vi "Diff_Drive_System_Act.vi"(6 "FPGA_Time_Seconds":dbl, 7 "Enabled":bool=TRUE, 9 "Right Speed":dbl, 10 "Left Speed":dbl, 11 "Diff_Drive_Device_Refs":T1 {"GyroDevRef"."Sample Rate" min=0.25 max=100.0 step=0.25}) -> ()   [LabVIEW 2019]
uses:
  <vilib>/Rock Robotics/WPI/ThirdParty/JAS_Junk/TrajLib/Trajectory_Library.lvlib
  Diff_Drive_System_Globals.vi
  <vilib>/Rock Robotics/SystemInterfaces/DIO/FPGA_DIOPWMChannel.ctl
  <vilib>/Rock Robotics/WPI/PWM/WPI_PWMDeadband.ctl
  <vilib>/Rock Robotics/WPI/MotorControl/WPI_MotorControlType.ctl
  <vilib>/Rock Robotics/SystemInterfaces/DIO/FPGA_DIOChannel.ctl
  <vilib>/Rock Robotics/WPI/MotorControl/WPI_MotorControlDeviceRef.ctl
  <vilib>/Rock Robotics/WPI/RobotDrive/WPI_RobotDriveDevRef.ctl
  <vilib>/Rock Robotics/SystemInterfaces/Encoder/FPGA_EncoderIdx.ctl
  <vilib>/Rock Robotics/WPI/Encoder/WPI_EncoderType.ctl
  <vilib>/Rock Robotics/SystemInterfaces/Counter/FPGA_CounterCtrSystemIndex.ctl
  <vilib>/Rock Robotics/WPI/Encoder/WPI_EncoderDevRef.ctl
  <vilib>/Rock Robotics/SystemInterfaces/spilib/spi_bus.ctl
  <vilib>/Rock Robotics/SystemInterfaces/AI/FPGA_AIChannel.ctl
  <vilib>/Rock Robotics/WPI/Gyro/WPI_GyroDevRef.ctl
  Diff_Drive_System_Device_Refs.ctl
panel:
  # "Analog"
  # "XRS"
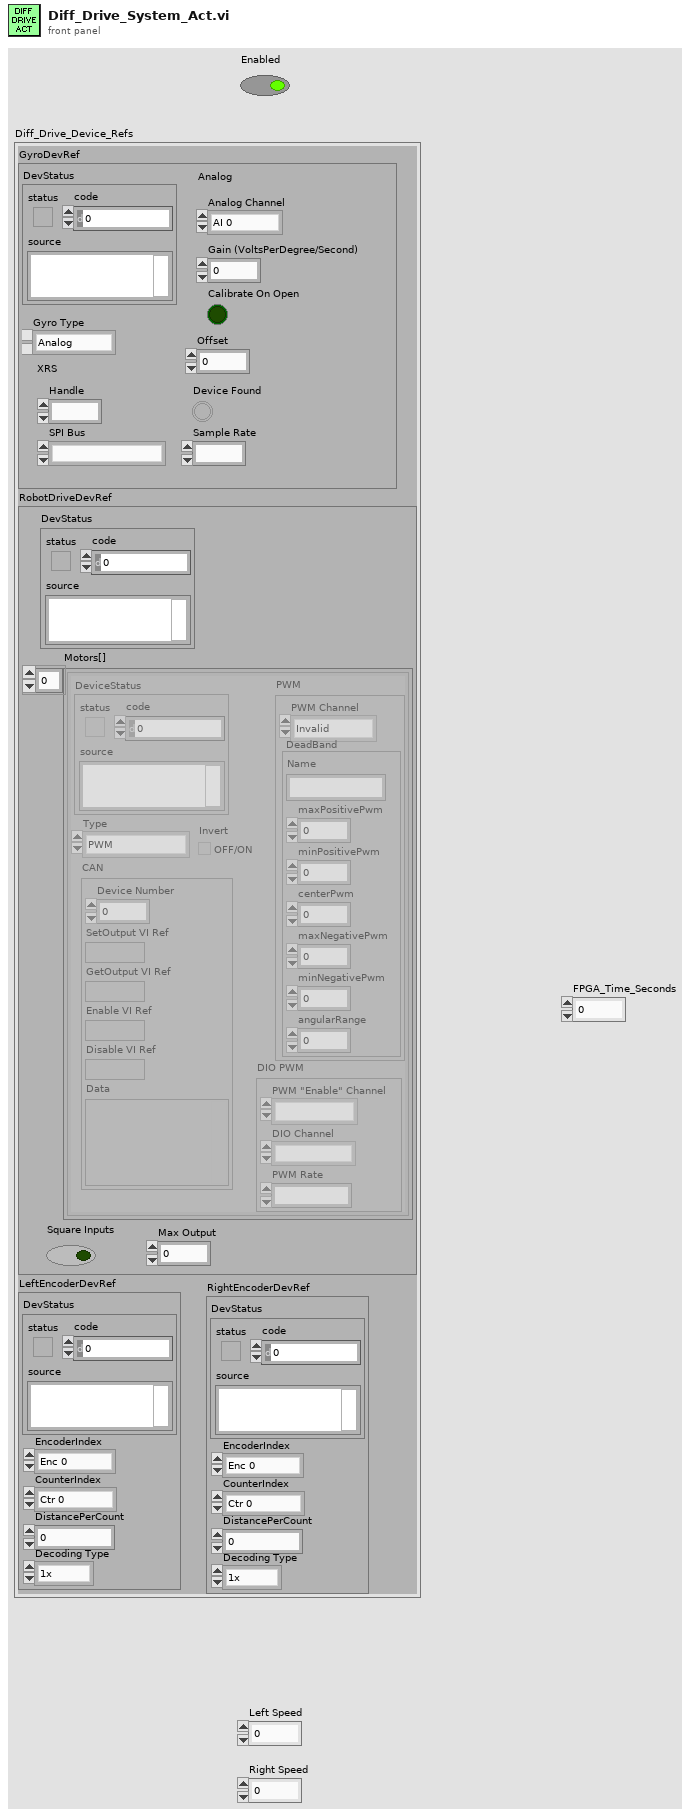
[diagram p1: front panel]
types:
  T1 = typedef "Diff_Drive_System_Device_Refs.ctl" = cluster{"GyroDevRef":T2, "RobotDriveDevRef":T5, "LeftEncoderDevRef":T11, "RightEncoderDevRef":T11}
  T2 = typedef "WPI_GyroDevRef.ctl" = cluster{"DevStatus":errorcluster, "Analog Channel":T3, "Gain (VoltsPerDegree/Second)":dbl, "Gyro Type":enum16{"Analog", "XRS450"}, "Handle":i32, "SPI Bus":T4, "Device Found":bool, "Sample Rate":dbl, "Calibrate On Open":bool, "Offset":dbl}
  T3 = typedef "FPGA_AIChannel.ctl" = enum8{"AI 0", "AI 1", "AI 2", "AI 3", "AI MXP 0", "AI MXP 1", "AI MXP 2", "AI MXP 3", "Invalid"}
  T4 = typedef "spi_bus.ctl" = enum16{"SPI On-Board, CS0", "SPI On-Board, CS1", "SPI On-Board, CS2", "SPI On-Board, CS3", "SPI MXP", "Invalid"}
  T5 = typedef "WPI_RobotDriveDevRef.ctl" = cluster{"DevStatus":errorcluster, "Motors[]":T6[], "Square Inputs":bool, "Max Output":dbl}
  T6 = typedef "WPI_MotorControlDeviceRef.ctl" = cluster{"DeviceStatus":errorcluster, "Type":T7, "PWM":cluster{"PWM Channel":T8, "DeadBand":T9}, "CAN":cluster{"Device Number":u8, "SetOutput VI Ref":variant, "GetOutput VI Ref":variant, "Enable VI Ref":variant, "Disable VI Ref":variant, "Data":variant}, "Invert":bool, "DIO PWM":cluster{"PWM \"Enable\" Channel":T8, "DIOChannel":T10, "PWM Rate":dbl}}
  T7 = typedef "WPI_MotorControlType.ctl" = enum16{"PWM", "CAN", "DIO PWM"}
  T8 = typedef "FPGA_DIOPWMChannel.ctl" = enum8{"PWM 0", "PWM 1", "PWM 2", "PWM 3", "PWM 4", "PWM 5", "PWM 6", "PWM 7", "PWM 8", "PWM 9", "PWM MXP 0", "PWM MXP 1", "PWM MXP 2", "PWM MXP 3", "PWM MXP 4", "PWM MXP 5", "PWM MXP 6", "PWM MXP 7", "PWM MXP 8", "PWM MXP 9", "Invalid"}
  T9 = typedef "WPI_PWMDeadband.ctl" = cluster{"Name":string, "maxPositivePwm":i32, "minPositivePwm":i32, "centerPwm":i32, "maxNegativePwm":i32, "minNegativePwm":i32, "angularRange":u16}
  T10 = typedef "FPGA_DIOChannel.ctl" = enum8{"DIO 0", "DIO 1", "DIO 2", "DIO 3", "DIO 4", "DIO 5", "DIO 6", "DIO 7", "DIO 8", "DIO 9", "DIO MXP 0", "DIO MXP 1", "DIO MXP 2", "DIO MXP 3", "DIO MXP 4", "DIO MXP 5", "DIO MXP 6", "DIO MXP 7", "DIO MXP 8", "DIO MXP 9", "DIO MXP 10", "DIO MXP 11", "DIO MXP 12", "DIO MXP 13", "DIO MXP 14", "DIO MXP 15", "SPI Port CS1", "SPI Port CS2", "SPI Port CS3", "SPI Port MISO", "SPI Port MOSI", "Invalid"}
  T11 = typedef "WPI_EncoderDevRef.ctl" = cluster{"DevStatus":errorcluster, "EncoderIndex":T12, "CounterIndex":T13, "DistancePerCount":dbl, "Decoding Type":T14}
  T12 = typedef "FPGA_EncoderIdx.ctl" = enum8{"Enc 0", "Enc 1", "Enc 2", "Enc 3", "Enc 4", "Enc 5", "Enc 6", "Enc 7", "Invalid"}
  T13 = typedef "FPGA_CounterCtrSystemIndex.ctl" = enum8{"Ctr 0", "Ctr 1", "Ctr 2", "Ctr 3", "Ctr 4", "Ctr 5", "Ctr 6", "Ctr 7", "Invalid"}
  T14 = typedef "WPI_EncoderType.ctl" = enum16{"1x", "2x", "4x"}
  T15 = typedef "Trajectory_Library.lvlib/SIMPLE_MOTOR_FF.ctl" = cluster{"Ks":dbl, "Kv":dbl, "Ka":dbl, "KnInv":dbl}
  T16 = typedef "Trajectory_Library.lvlib/PID_ADV_LIMITS.ctl" = cluster{"MaxInput":dbl, "MinInput":dbl, "Continuous":bool, "MaxOutput":dbl, "MinOutput":dbl}
  T17 = typedef "Trajectory_Library.lvlib/PID_ADV_TUNING.ctl" = cluster{"Kf":dbl, "Kp":dbl, "Ki":dbl, "Kd":dbl, "MaximumIntegral":dbl, "MinimumIntegral":dbl, "Filter Derivative":bool}
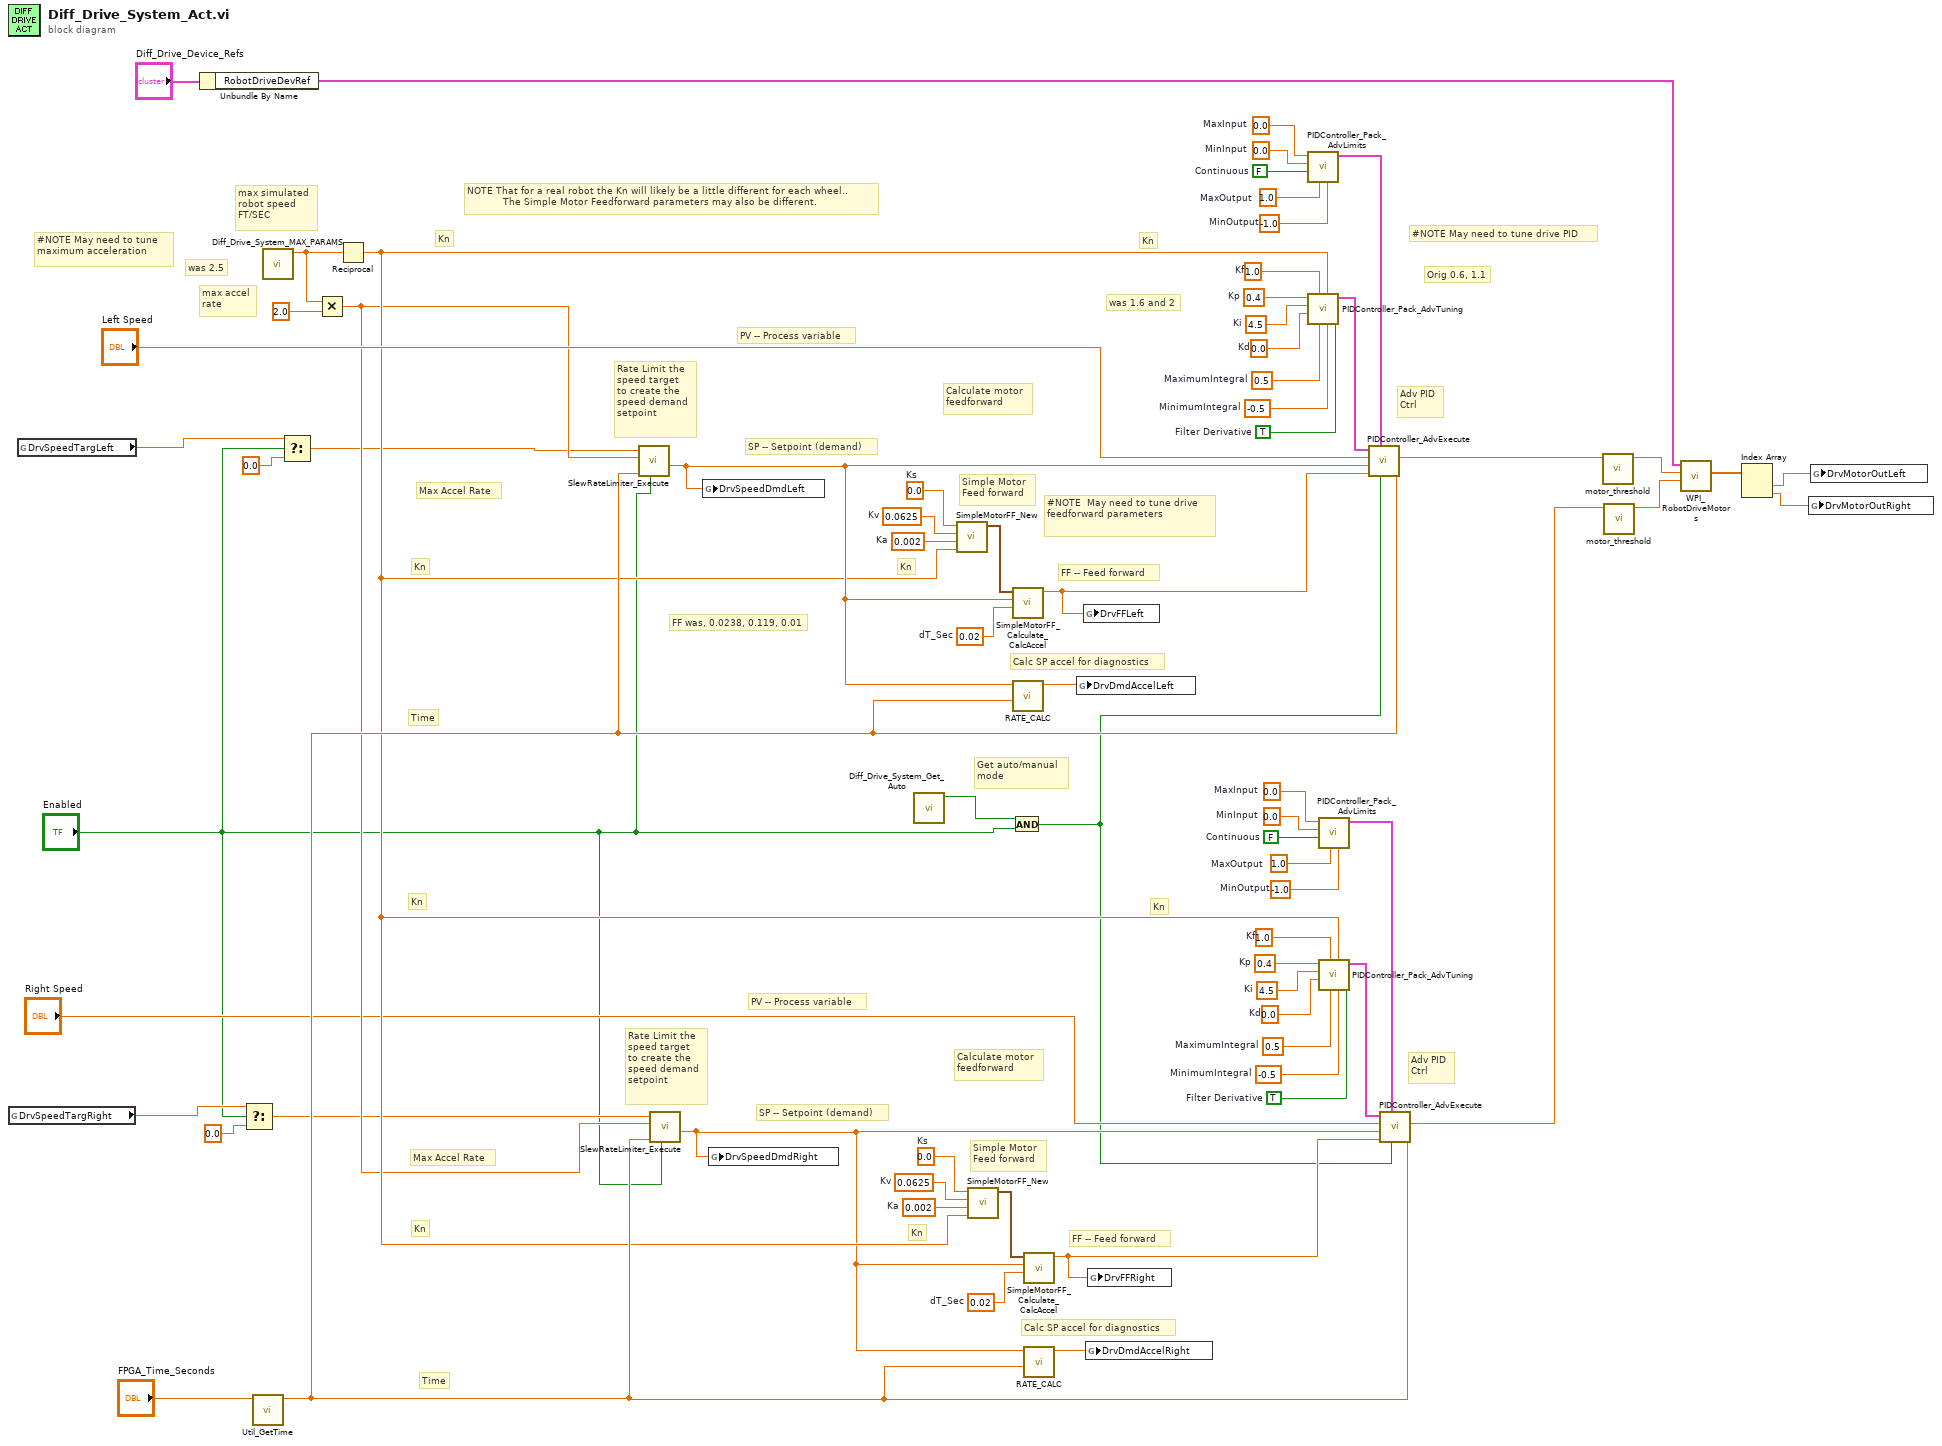
[diagram p0: block diagram]
diagram:
  w31 = 0.4  # Kp
  w30 = 4.5  # Ki
  w29 = 0.0  # Kd
  w28 = 1.0  # Kf
  w27 = 0.5  # MaximumIntegral
  w26 = -0.5  # MinimumIntegral
  w25 = TRUE  # Filter Derivative
  w23 = 0.0  # MinInput
  w22 = FALSE  # Continuous
  w21 = 1.0  # MaxOutput
  w24 = -1.0  # MinOutput
  w20 = 0.0  # MaxInput
  w36 = 0.02  # dT_Sec
  w34 = 0.0  # Ks
  w33 = 0.0625  # Kv
  w32 = 0.002  # Ka
  w56 = 0.4  # Kp
  w55 = 4.5  # Ki
  w54 = 0.0  # Kd
  w53 = 1.0  # Kf
  w52 = 0.5  # MaximumIntegral
  w51 = -0.5  # MinimumIntegral
  w50 = TRUE  # Filter Derivative
  w48 = 0.0  # MinInput
  w47 = FALSE  # Continuous
  w46 = 1.0  # MaxOutput
  w49 = -1.0  # MinOutput
  w45 = 0.0  # MaxInput
  w61 = 0.02  # dT_Sec
  w59 = 0.0  # Ks
  w58 = 0.0625  # Kv
  w57 = 0.002  # Ka
  # "was 1.6 and 2"
  # "Get auto/manual\nmode"
  # "FF was, 0.0238, 0.119, 0.01"
  # "Orig 0.6, 1.1"
  # "NOTE That for a real robot the Kn will likely be a little different for each wheel..\n            The Simple Motor Feedforward parameters may also be different."
  # "Max Accel Rate"
  # "Max Accel Rate"
  # "Time"
  # "Kn"
  # "Kn"
  # "Kn"
  # "Kn"
  # "Time"
  # "Kn"
  # "PV -- Process variable"
  # "Kn"
  # "Calc SP accel for diagnostics"
  # "FF -- Feed forward"
  # "SP -- Setpoint (demand)"
  # "Adv PID\nCtrl"
  # "Calculate motor\nfeedforward"
  # "Rate Limit the \nspeed target\nto create the\nspeed demand\nsetpoint"
  # "Simple Motor\nFeed forward"
  # "Kn"
  # "PV -- Process variable"
  # "Kn"
  # "Calc SP accel for diagnostics"
  # "FF -- Feed forward"
  # "SP -- Setpoint (demand)"
  # "Adv PID\nCtrl"
  # "Calculate motor\nfeedforward"
  # "was 2.5"
  # "Rate Limit the \nspeed target\nto create the\nspeed demand\nsetpoint"
  # "Simple Motor\nFeed forward"
  # "#NOTE May need to tune drive PID"
  # "#NOTE May need to tune maximum acceleration"
  # "#NOTE  May need to tune drive feedforward parameters"
  # "max simulated\nrobot speed\nFT/SEC"
  # "max accel\nrate"
  n1 = global read "Diff_Drive_System_Globals.vi" "DrvSpeedTargRight"() -> (w7:dbl)
  n2 = global read "Diff_Drive_System_Globals.vi" "DrvSpeedTargLeft"() -> (w3:dbl)
  n3 = Unbundle By Name("Diff_Drive_Device_Refs") -> ("RobotDriveDevRef"=w64:T5)
  n4 = Select(t=w7, s="Enabled", f=0.0) -> (s? t:f=w5:dbl)
  n5 = call <vilib>:"Util_GetTime.vi"("Pass_Through_Time"="FPGA_Time_Seconds") -> ("FPGA_Time_Seconds"=w16:dbl)  [unwired: 9 in, 1 out]
  n6 = call "Diff_Drive_System_MAX_PARAMS.vi"() -> ("Max Speed Ft/Sec"=w40:dbl)  [unwired: 9 in, 2 out]
  n7 = Select(t=w3, s="Enabled", f=0.0) -> (s? t:f=w2:dbl)
  n8 = Multiply(x=w40, y=2.0 ("x")) -> (x*y=w14:dbl)
  n9 = Reciprocal(x=w40) -> (1/x=w15:dbl)
  n10 = call <vilib>:"SlewRateLimiter_Execute.vi"("Enable"="Enabled", "Time"=w16, "PositiveRate"=w14, "Input"=w2) -> ("Output"=w42:dbl)  [unwired: 6 in, 1 out]
  n11 = call <vilib>:"SlewRateLimiter_Execute.vi"("Enable"="Enabled", "Time"=w16, "PositiveRate"=w14, "Input"=w5) -> ("Output"=w10:dbl)  [unwired: 6 in, 1 out]
  n12 = global write "Diff_Drive_System_Globals.vi" "DrvSpeedDmdLeft"(w42) -> ()
  n13 = global write "Diff_Drive_System_Globals.vi" "DrvSpeedDmdRight"(w10) -> ()
  n14 = call "Diff_Drive_System_Get_Auto.vi"() -> ("Auto Mode"=w9:bool)  [unwired: 11 in]
  n15 = call <vilib>:"SimpleMotorFF_New.vi"("Kn"=w15, "Ka"=w57, "Kv"=w58, "Ks"=w59) -> ("SIMPLE_MOTOR_FF"=w60:T15)  [unwired: 7 in]
  n16 = call <vilib>:"SimpleMotorFF_New.vi"("Kn"=w15, "Ka"=w32, "Kv"=w33, "Ks"=w34) -> ("SIMPLE_MOTOR_FF"=w35:T15)  [unwired: 7 in]
  n17 = And(x=w9, y="Enabled") -> (x .and. y?=w8:bool)
  n18 = call <vilib>:"SimpleMotorFF_Calculate_CalcAccel.vi"("dT_Sec"=w61, "VelSp"=w42, "SIMPLE_MOTOR_FF"=w60) -> ("FeedForward"=w39:dbl)  [unwired: 8 in]
  n19 = call "RATE_CALC.vi"("Time"=w16, "Input"=w42) -> ("Output"=w41:dbl)  [unwired: 9 in]
  n20 = call <vilib>:"SimpleMotorFF_Calculate_CalcAccel.vi"("dT_Sec"=w36, "VelSp"=w10, "SIMPLE_MOTOR_FF"=w35) -> ("FeedForward"=w12:dbl)  [unwired: 8 in]
  n21 = call "RATE_CALC.vi"("Time"=w16, "Input"=w10) -> ("Output"=w11:dbl)  [unwired: 9 in]
  n22 = global write "Diff_Drive_System_Globals.vi" "DrvDmdAccelLeft"(w41) -> ()
  n23 = global write "Diff_Drive_System_Globals.vi" "DrvFFLeft"(w39) -> ()
  n24 = global write "Diff_Drive_System_Globals.vi" "DrvDmdAccelRight"(w11) -> ()
  n25 = global write "Diff_Drive_System_Globals.vi" "DrvFFRight"(w12) -> ()
  n26 = call <vilib>:"PIDController_Pack_AdvLimits.vi"("MinOutput"=w49, "MaxOutput"=w46, "Continuous"=w47, "MinInput"=w48, "MaxInput"=w45) -> ("Adv PID Limits"=w43:T16)  [unwired: 6 in]
  n27 = call <vilib>:"PIDController_Pack_AdvTuning.vi"("Filter Derivative"=w50, "MinimumIntegral"=w51, "Kn"=w15, "MaximumIntegral"=w52, "Kf"=w53, "Kd"=w54, "Ki"=w55, "Kp"=w56) -> ("Adv PID Tuning"=w44:T17)  [unwired: 3 in]
  n28 = call <vilib>:"PIDController_Pack_AdvLimits.vi"("MinOutput"=w24, "MaxOutput"=w21, "Continuous"=w22, "MinInput"=w23, "MaxInput"=w20) -> ("Adv PID Limits"=w18:T16)  [unwired: 6 in]
  n29 = call <vilib>:"PIDController_Pack_AdvTuning.vi"("Filter Derivative"=w25, "MinimumIntegral"=w26, "Kn"=w15, "MaximumIntegral"=w27, "Kf"=w28, "Kd"=w29, "Ki"=w30, "Kp"=w31) -> ("Adv PID Tuning"=w19:T17)  [unwired: 3 in]
  n30 = call <vilib>:"PIDController_AdvExecute.vi"("Time"=w16, "Auto"=w8, "Adv PID Limits"=w43, "FF-FeedForward"=w39, "SP-SetPoint"=w42, "PV-Measurement"="Left Speed", "Adv PID Tuning"=w44) -> ("CO-ControlOutput"=w38:dbl)  [unwired: 2 in, 2 out]
  n31 = call <vilib>:"PIDController_AdvExecute.vi"("Time"=w16, "Auto"=w8, "Adv PID Limits"=w18, "FF-FeedForward"=w12, "SP-SetPoint"=w10, "PV-Measurement"="Right Speed", "Adv PID Tuning"=w19) -> ("CO-ControlOutput"=w17:dbl)  [unwired: 2 in, 2 out]
  n32 = call "motor_threshold.vi"("motor in"=w38) -> ("motor out"=w68:dbl)  [unwired: 10 in]
  n33 = call "motor_threshold.vi"("motor in"=w17) -> ("motor out"=w69:dbl)  [unwired: 10 in]
  n34 = call <vilib>:"WPI_RobotDriveMotors.vi"("RightSpeed"=w69, "LeftSpeed"=w68, "RobotDriveDevRef"=w64) -> ("Motor Values"=w67:dbl[])  [unwired: 6 in, 2 out]
  n35 = Index Array(array=w67) -> (element #1=w63:dbl, element #2=w62:dbl)  [unwired: 2 in]
  n36 = global write "Diff_Drive_System_Globals.vi" "DrvMotorOutRight"(w62) -> ()
  n37 = global write "Diff_Drive_System_Globals.vi" "DrvMotorOutLeft"(w63) -> ()
